vi "Render_Frame.vi"(0 "Channels":T3, 1 "Memory":T1={"RoomKey"=-1, "Key"=-1, "NameKey"=-1, "Lit"=[], "Dim"=[], "Dark"=[], "Comp"=[], "Template"={"image type"=0, "image depth"=0, "image"=[], "mask"=[], "colors"=[], "Rectangle"={"left"=0, "top"=0, "right"=0, "bottom"=0}}, "CX"=-1, "CY"=-1, "X1"=0, "Y1"=0, "X2"=0, "Y2"=0, "Prev"=[], "HudKey"=-1, "HudScore"=-1, "HudTime"=-1, "Full"=[]}, 2 "Last ms":u32, 5 "Sprites":cluster{"Pix":u8[][], "Mask":u8[][]}[](array[cluster]), 7 "Hud":T2, 9 "Title":T2, 11 "error in":errorcluster) -> (4 "Picture":picture, 6 "Memory out":T1={"RoomKey"=-1, "Key"=-1, "NameKey"=-1, "Lit"=[], "Dim"=[], "Dark"=[], "Comp"=[], "Template"={"image type"=0, "image depth"=0, "image"=[], "mask"=[], "colors"=[], "Rectangle"={"left"=0, "top"=0, "right"=0, "bottom"=0}}, "CX"=-1, "CY"=-1, "X1"=0, "Y1"=0, "X2"=0, "Y2"=0, "Prev"=[], "HudKey"=-1, "HudScore"=-1, "HudTime"=-1, "Full"=[]}, 8 "FPS":dbl, 10 "Now ms":u32, 13 "Stop":bool, 14 "Tick":i32, 15 "error out":errorcluster)   [LabVIEW 2020, in "GH_App.lvlib"]
doc: "One frame: waits (at most 200 ms) for the next game state and draws it with Frame_Draw. Without a new state nothing is drawn and Memory stays. FPS from the time since the last frame. Stop on Quit or on an error."
uses:
  GH_App.lvlib
  Render/GH_Render.lvlib
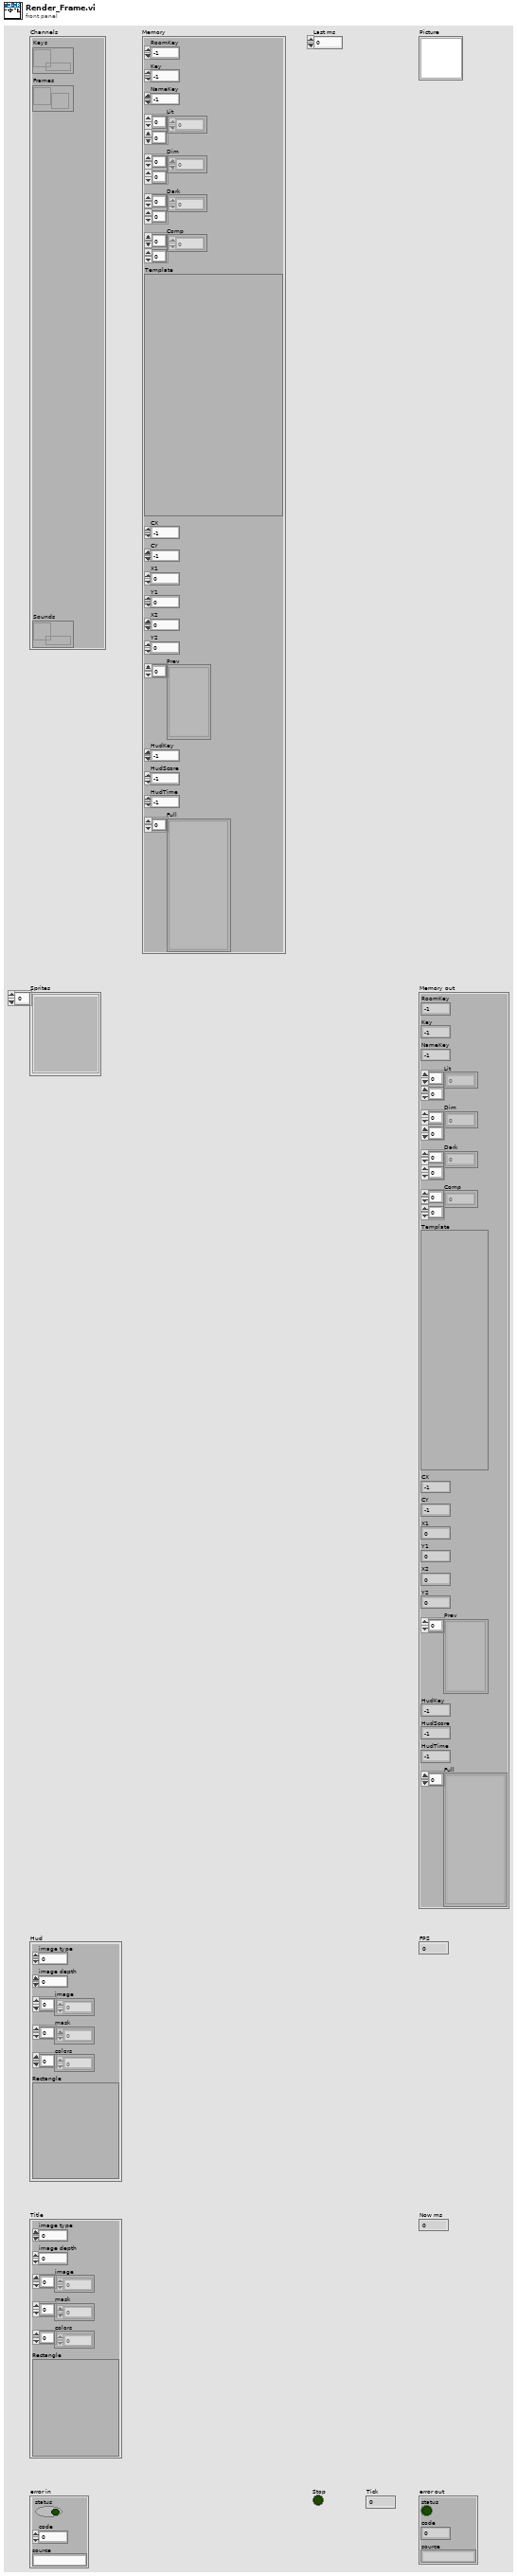
[diagram p1: front panel]
types:
  T1 = cluster{"RoomKey":i32, "Key":i32, "NameKey":i32, "Lit":u8[][], "Dim":u8[][], "Dark":u8[][], "Comp":u8[][], "Template":cluster{"image type":i32, "image depth":i32, "image":u8[], "mask":u8[], "colors":u32[], "Rectangle":cluster{"left":i16, "top":i16, "right":i16, "bottom":i16}}, "CX":i32, "CY":i32, "X1":i32, "Y1":i32, "X2":i32, "Y2":i32, "Prev":cluster{"Kind":i32, "X10":i32, "Y10":i32, "Dir":i32, "Mode":i32}[], "HudKey":i32, "HudScore":i32, "HudTime":i32, "Full":cluster{"image type":i32, "image depth":i32, "image":u8[], "mask":u8[], "colors":u32[], "Rectangle":cluster{"left":i16, "top":i16, "right":i16, "bottom":i16}}[]}
  T2 = cluster{"image type":i32, "image depth":i32, "image":u8[], "mask":u8[], "colors":u32[], "Rectangle":cluster{"left":i16, "top":i16, "right":i16, "bottom":i16}}
  T3 = cluster{"Keys":refnum<queue>, "Frames":refnum<notifier>, "Sounds":refnum<queue>}
  T4 = cluster{"Tick":u32, "Phase":i32, "PhaseTicks":i32, "Level":i32, "Room":i32, "X10":i32, "Y10":i32, "VY10":i32, "Mode":i32, "Facing":i32, "Run":i32, "Vert":i32, "StandY":i32, "EntryX10":i32, "EntryY10":i32, "EntryMode":i32, "Lives":i32, "Score":i32, "NextLife":i32, "KeyR":i32, "KeyB":i32, "KeyY":i32, "Torch":bool, "FloorPhase":i32, "Dead":bool, "LevelStart":bool, "Quit":bool, "Sound":i32, "Seed":u32, "DemoStep":i32, "Tiles":u8[][], "World":cluster{"ID":string, "Depth":i32, "Column":i32, "Tiles":u8[][]}[], "Enemies":cluster{"Kind":i32, "X10":i32, "Y10":i32, "Dir":i32, "Mode":i32}[], "Highscores":cluster{"Score":i32, "Name":string}[], "Name":i32[], "Cursor":i32}
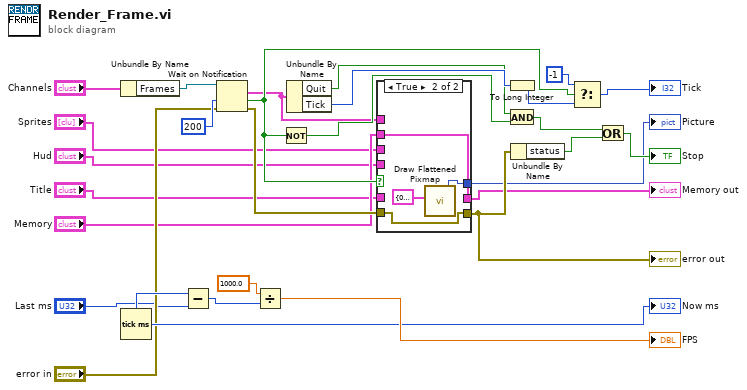
[diagram p0: block diagram]
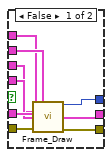
[diagram p2: hidden frame]
diagram:
  n1 = Unbundle By Name("Channels") -> ("Frames"=w8:refnum<notifier>)
  n2 = Tick Count (ms)() -> (millisecond timer value=w18:u32)
  "Now ms" <- w18
  n3 = Subtract(x=w18, y="Last ms") -> (x-y=w20:u32)
  n4 = Wait on Notification(notifier=w8, timeout in ms (-1)=200 ("Timeout"), error in (no error)="error in") -> (notification=w10:T4, timed out?=w11:bool, error out=w12:errorcluster)  [unwired: 1 in, 1 out]
  n5 = Divide(x=1000.0, y=w20) -> (x/y=→"FPS":dbl)
  n6 = Not(x=w11) -> (.not. x?=w25:bool)
  n7 = Unbundle By Name(w10) -> ("Quit"=w16:bool, "Tick"=w17:u32)
  n8 = case shown="True" w11 {
    tunnel: "Sprites" -> [w30 _]
    tunnel: "Hud" -> [w31 _]
    tunnel: "Title" -> [w32 _]
    tunnel: "Memory" -> [w33 w38]
    tunnel: w10 -> [w29 _]
    tunnel: w12 -> [w34 w39]
    tunnel: [w35 w41] -> w13
    tunnel: [w36 w38] -> w14
    tunnel: [w37 w39] -> w15
    frame False {
      n9 = call "Frame_Draw.vi"("State"=w29, "Memory"=w33, "Sprites"=w30, "Hud"=w31, "Title"=w32, "error in"=w34) -> ("Picture"=w35:picture, "Memory out"=w36:T1, "error out"=w37:errorcluster)  [unwired: 6 in, 1 out]
    }
    frame True {
      n10 = call <vilib>:"Draw Flattened Pixmap.vi"("image data"=T2 {"image type"=0, "image depth"=0, "image"=[], "mask"=[], "colors"=[], "Rectangle"={"left"=0, "top"=0, "right"=0, "bottom"=0}} ("No pixels")) -> ("new picture"=w41:picture)  [unwired: 8 in]
    }
  }
  "Picture" <- w13
  "Memory out" <- w14
  "error out" <- w15
  n11 = To Long Integer(number=w17) -> (32bit integer=w23:i32)
  n12 = And(x=w16, y=w25) -> (x .and. y?=w26:bool)
  n13 = Unbundle By Name(w15) -> ("status"=w27:bool)
  n14 = Select(t=-1, s=w11, f=w23) -> (s? t:f=→"Tick":i32)
  n15 = Or(x=w26, y=w27) -> (x .or. y?=→"Stop":bool)
